vi "CSE routine - Remove non-unique strings.vi"(5 "case sensitive comparison (T)":bool=TRUE, 6 "error in":errorcluster, 9 "Array in":string[](array[string])) -> (0 "error out":errorcluster, 3 "Array out":string[](array[string]))   [LabVIEW 2021]
doc: "The VI removes duplicated (non-unique) strings from a string array.\n\n::: CalcExpress Toolkit :::\nCopyright (c) 2000-2026 Konstantin Shifershteyn. All rights reserved."
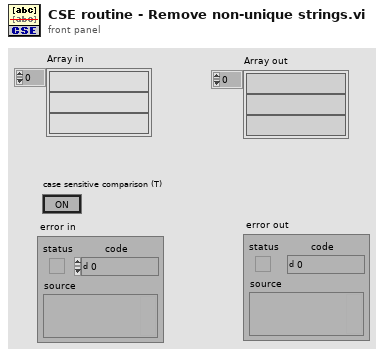
[diagram p1: front panel]
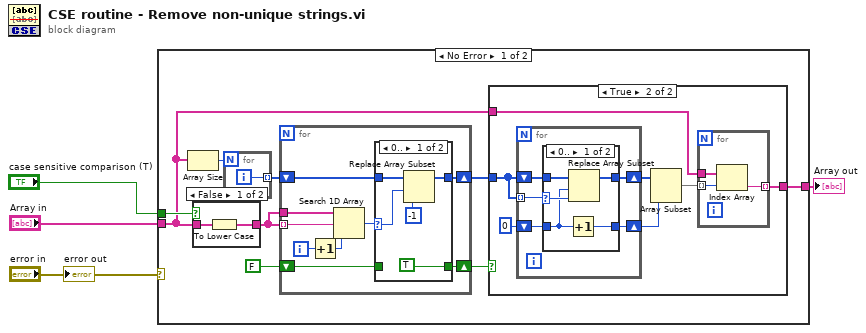
[diagram p0: block diagram]
diagram:
  n1 = case shown="No Error" "error in" {
    tunnel: "case sensitive comparison (T)" -> [w11 _]
    tunnel: [w10 w57] -> w3
    tunnel: "Array in" -> [w8 w57]
    frame No Error {
      n2 = Array Size(array=w8) -> (size(s)=w9:i32)
      n3 = case shown="False" w11 {
        tunnel: [w38 w39] -> w12
        tunnel: w8 -> [w37 w39]
        frame False {
          n4 = To Lower Case(string=w37) -> (all lower case string=w38:string[])
        }
        frame True {
        }
      }
      n5 = for {
        N: w9 -> [_]
        tunnel: [w56] -> w13 mode=indexing
        i -> [w56]
      }
      n6 = for {
        shift-right: [w43] -> w7
        shift-left: w13 -> [w44]
        tunnel: w12 -> [w48] mode=indexing
        tunnel: w12 -> [w47]
        shift-right: [w40] -> w5
        shift-left: FALSE -> [w41]
        i -> [w42]
        n7 = Increment(x=w42) -> (x+1=w46:i32)
        n8 = Search 1D Array(1D array=w47, element=w48, start index (0)=w46) -> (index of element=w45:i32)
        n9 = case shown="0.." w45 {
          selector: w45 -> [w52 _]
          tunnel: w44 -> [w53 w55]
          tunnel: [w51 w55] -> w43
          tunnel: w41 -> [_ w54]
          tunnel: [TRUE w54] -> w40
          frame 0.. {
            n10 = Replace Array Subset(array=w53, new element=-1 ("new element/subarray"), index=w52) -> (w51:i32[])
          }
          frame ..-1 {
          }
        }
      }
      n11 = case shown="True" w5 {
        tunnel: [w14 w17] -> w10
        tunnel: w8 -> [w14 w16]
        tunnel: w7 -> [_ w15]
        frame False {
        }
        frame True {
          n12 = for {
            shift-right: [w27] -> w20
            shift-left: w15 -> [w28]
            tunnel: w15 -> [w29] mode=indexing
            shift-right: [w25] -> w19
            shift-left: 0 -> [w26]
            n13 = case shown="0.." w29 {
              selector: w29 -> [w31 _]
              tunnel: w28 -> [w33 w36]
              tunnel: [w32 w36] -> w27
              tunnel: w26 -> [w30 w35]
              tunnel: [w34 w35] -> w25
              frame 0.. {
                n14 = Increment(x=w30) -> (x+1=w34:i32)
                n15 = Replace Array Subset(array=w33, new element=w31, index=w30) -> (w32:i32[])
              }
              frame ..-1 {
              }
            }
          }
          n16 = Array Subset(array=w20, length=w19) -> (w18:i32[])  [unwired: 1 in]
          n17 = for {
            tunnel: w18 -> [w24] mode=indexing
            tunnel: w16 -> [w23]
            tunnel: [w22] -> w17 mode=indexing
            n18 = Index Array(array=w23, index=w24) -> (element=w22:string)
          }
        }
      }
    }
    frame Error {
    }
  }
  "Array out" <- w3
  "error out" <- "error in"
